vi "RCtest.vi"(8 "error in (no error)":errorcluster, 11 "s":bool) -> (0 "error out":errorcluster)   [LabVIEW 2019]
uses:
  <vilib>/myRIO/Instrument Drivers/Onboard IO/PWM/typedefs/PWM Reference.ctl
  <vilib>/myRIO/Common/Instrument Driver Framework/Utilities/typedefs/myRIO Generic Hardware Reference.ctl
  <vilib>/myRIO/Common/Instrument Driver Framework/Utilities/typedefs/Hardware Version Enum.ctl
  <vilib>/myRIO/Common/Instrument Driver Framework/Utilities/typedefs/myRIO v1.0 Reference.ctl
  <vilib>/myRIO/Common/Instrument Driver Framework/Utilities/typedefs/Generic FPGA Reference.ctl
  <vilib>/myRIO/Common/Instrument Driver Framework/myRIO v1.0/PWM/typedefs/PWM Channels Enum.ctl
  <vilib>/myRIO/Instrument Drivers/Onboard IO/PWM/typedefs/PWM Configuration.ctl
  <vilib>/userDefined/High Color/nirio_resource_hc.ctl
  <vilib>/myRIO/Common/Instrument Driver Framework/Utilities/vis/Is FPGA Ref Available.vi
  <vilib>/myRIO/Common/Instrument Driver Framework/myRIO v1.0/PWM/vis/myRIO v1.1 Open PWM.vi
  <vilib>/myRIO/Instrument Drivers/Onboard IO/PWM/vis/Set Duty Cycle and Frequency.vi
  <vilib>/myRIO/Common/Instrument Driver Framework/Utilities/vis/Validate Channels.vi
  <vilib>/myRIO/Common/Instrument Driver Framework/myRIO v1.0/PWM/vis/myRIO v1.0 Reserve PWM.vi
  <vilib>/myRIO/Common/Instrument Driver Framework/myRIO v1.0/PWM/vis/myRIO v1.0 Build MUX Configuration PWM.vi
  <vilib>/myRIO/Common/Instrument Driver Framework/myRIO v1.0/Resource Manager/vis/myRIO v1.0 Reserve Channel List.vi
  <vilib>/myRIO/Common/Instrument Driver Framework/myRIO v1.0/Resource Manager/vis/myRIO v1.0 Create Configuration List.vi
  <vilib>/myRIO/Common/Instrument Driver Framework/myRIO v1.0/Resource Manager/vis/myRIO v1.0 Reserve Channel.vi
  <vilib>/myRIO/Common/Instrument Driver Framework/myRIO v1.0/Resource Manager/vis/myRIO v1.0 Unreserve Channel.vi
  <vilib>/myRIO/Common/Instrument Driver Framework/myRIO v1.0/Resource Manager/vis/myRIO v1.0 Build Mutex Name.vi
  <vilib>/Utility/VariantDataType/GetNumericInfo.vi
  <vilib>/Utility/error.llb/Error Cluster From Error Code.vi
  <vilib>/myRIO/Common/Instrument Driver Framework/myRIO v1.0/myRIO v1.1 Open.vi
  <vilib>/myRIO/Common/Instrument Driver Framework/Utilities/vis/IO Manager.vi
  <vilib>/myRIO/Common/Instrument Driver Framework/Utilities/vis/Configuration Manager.vi
  <vilib>/myRIO/Common/Instrument Driver Framework/myRIO v1.0/Resource Manager/vis/myRIO v1.0 Configure IO.vi
  <vilib>/myRIO/Common/Instrument Driver Framework/myRIO v1.0/myRIO v1.0 Close.vi
  <vilib>/myRIO/Common/Instrument Driver Framework/myRIO v1.0/PWM/vis/myRIO v1.0 Write PWM.vi
  <vilib>/myRIO/Express VI/Onboard IO/PWM/PWM Express VI.xnode
  <vilib>/myRIO/Instrument Drivers/Onboard IO/PWM/vis/myRIO PWM Open.xnode
  <vilib>/myRIO/Instrument Drivers/Onboard IO/PWM/PWM.lvlib
panel:
  in  "upper limit":dbl=0.125 format="%#_13g"
  in  "lower limit":dbl=0.02 format="%#_13g"
  in  "f":dbl=180.0
  in  "x":dbl=65.0
  # "T§¨\nF¶}"
  # "0.02~0.125"
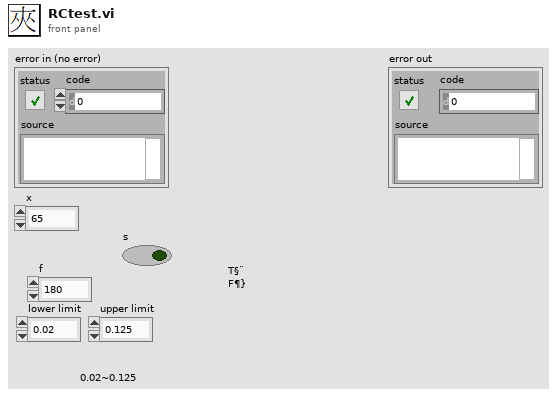
[diagram p1: front panel]
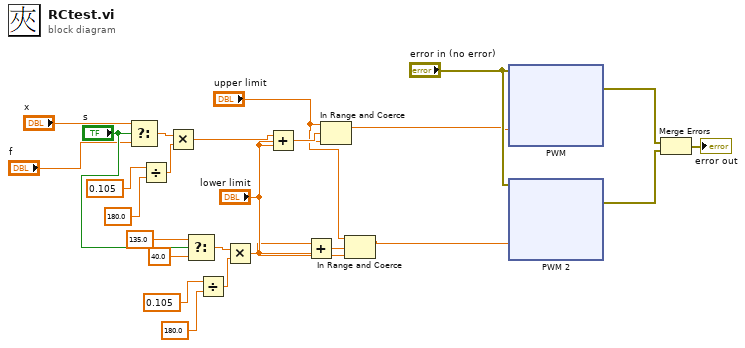
[diagram p0: block diagram]
diagram:
  n1 = Select(t="x", s="s", f="f") -> (s? t:f=w21:dbl)
  n2 = Divide(x=0.105 ("y"), y=180.0 ("x")) -> (x/y=w18:dbl)
  n3 = Multiply(x=w21, y=w18) -> (x*y=w15:dbl)
  n4 = Select(t=135.0, s="s", f=40.0) -> (s? t:f=w9:dbl)
  n5 = Divide(x=0.105 ("y"), y=180.0 ("x")) -> (x/y=w11:dbl)
  n6 = Multiply(x=w9, y=w11) -> (x*y=w8:dbl)
  n7 = Add(x=w15, y="lower limit") -> (x+y=w16:dbl)
  n8 = Add(x=w8, y="lower limit") -> (x+y=w13:dbl)
  n9 = In Range and Coerce(upper limit="upper limit", x=w16, lower limit="lower limit") -> (coerced(x)=w17:dbl)  [unwired: 1 out]
  n10 = In Range and Coerce(upper limit="upper limit", x=w13, lower limit="lower limit") -> (coerced(x)=w14:dbl)  [unwired: 1 out]
  n11 = xnode "PWM"("Duty Cycle"=w17, "error in (no error)"="error in (no error)") -> ("error out"=w24:errorcluster)
  n12 = xnode "PWM 2"("Duty Cycle"=w14, "error in (no error)"="error in (no error)") -> ("error out"=w23:errorcluster)
  n13 = Merge Errors(w24, w23) -> (→"error out":errorcluster)
